vi "DialogCreateInterface.vi"(0 "ClassWriterNative.lvclass":refnum<class "ClassWriterNative.lvclass">, 1 "ProjectItem Refnum":refnum<vi>, 5 "error in (no error)":errorcluster) -> (14 "Reference out":refnum<class "ClassWriterNative.lvclass">, 15 "Cancelled":bool, 16 "CreateInterfaceData":T3, 19 "error out":errorcluster)   [LabVIEW 2020, in "ClassWriterNative.lvclass"]
uses:
  ClassWriterNative.lvclass
  Provider_BaseClassInterface/CreateInterfaceData.ctl
  Provider_BaseClassInterface/ClassWriter_class/InterfaceMethodsToCreate.ctl
  Common/CommonVIs/CommonVIs_AttributeType.ctl
  Common/CommonVIs/CommonVIs_AttributeDataType.ctl
  Common/String/GDSString_AccessScopeModifierType.ctl
  Provider_BaseClassInterface/BaseProvider_SubVIs/BaseProvider_WireList.ctl
  Provider_BaseClassInterface/BaseProvider_SubVIs/BaseProvider_WireStyleType.ctl
  <vilib>/Utility/miscctls.llb/LVRectTypeDef.ctl
  Common/InterfaceLibrary/InterfaceInfo.ctl
  Common/LvClass_class/GDSLvClass_ClassMethodInfo.ctl
  Common/CommonVIs/CommonVIs_ClassIconSelection_Action.ctl
  <vilib>/Utility/miscctls.llb/LVPositionTypeDef.ctl
  <vilib>/Utility/miscctls.llb/LVRowAndColumnUnsignedTypeDef.ctl
  <vilib>/picture/picture.llb/imagedata.ctl
  8226ef7b-d77c-4b82-be33-8974597c5039.vi
  914e6089-59b2-486e-920a-8b2175e33088.vi
  Common/InterfaceLibrary/InterfaceLibrary.lvlib
  Provider_BaseClassInterface/ClassWriter_class/ClassWriter.lvclass
panel:
  out "IconSelection":picture
  in  "WireSelectionList":T1
  out "Wire Style":cluster{"Name":string, "Wire":picture}
  in  "InterfaceFilter":string caption="Filter"
  out "Icon":picture
  in  "_ShowContextHelp":bool
  in  "Help":bool
  in  "ConnectorPanePattern":u16(ring) caption="Connector Pane" items=["4x4x4", "5x6x5", "6x8x6"]
  in  "_UseLLB":bool
  in  "_InterfaceFolderSuffix":string caption="Interface Folder Suffix"
  out "ProductPicture":picture
  out "DupPath":bool
  in  "_InterfaceName":string caption="Interface Name"
  in  "_ClassDescription":string caption="Interface Description"
  in  "_InterfaceFolder":path caption="Save Interface To.."
  out "TriggerSuffixChange":string
  in  "SelectInterfaceClass":i32[](listbox) caption="Select Parent Interface(s) (ctrl+click to do multiple Selection)"
  in  "M":string[][](table)
  out "Over":i32(listbox) caption="Over\nride?"
  out "IconList":i32(listbox)
  in  "Cancel":bool
  in  "CreateInterface":bool
  # "Icon"
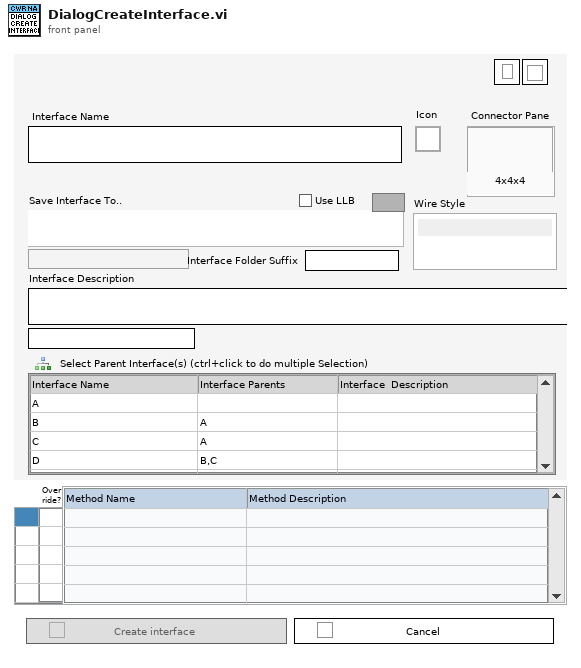
[diagram p1: front panel]
types:
  T1 = typedef "BaseProvider_WireList.ctl" = cluster{"WireStyle":T2[], "WireEditor":bool}
  T2 = typedef "BaseProvider_WireStyleType.ctl" = cluster{"Boolean":bool, "Wire":picture, "Name":string, "Status":u16}
  T3 = typedef "ClassWriter.lvclass/CreateInterfaceData.ctl" = cluster{"InterfaceName":string, "InterfaceFolder":path, "InterfaceDescription":string, "FolderSuffix":string, "MethodsToCreate":T4[], "ParentInterfaces":path[]}
  T4 = typedef "ClassWriter.lvclass/InterfaceMethodsToCreate.ctl" = cluster{"Name":string, "Description":string, "MethodsArgumentsIn":T5[], "MethodsArgumentsOut":T5[], "DecendantsMustOverride":bool}
  T5 = typedef "CommonVIs_AttributeType.ctl" = cluster{"Name":string, "DataType":T6, "ArrayDim":i32, "CtrlPath":path, "DataTypeString":string, "AccessScope":T7, "InitialData":variant}
  T6 = typedef "CommonVIs_AttributeDataType.ctl" = enum16{"UINT8", "INT8", "UINT16", "INT16", "UINT32", "INT32", "UINT64", "INT64", "SGL", "DBL", "EXT", "CSG", "CDB", "CXT", "TimeStamp", "STRING", "PATH", "BOOL", "ENUM", "RefNum", "VIRefNum", "LabVIEW Class", "Cluster", "Variant", "TypeDef", "Waveform", "LabVIEW Object", "Other", "void", "Set", "Map"}
  T7 = typedef "GDSString_AccessScopeModifierType.ctl" = enum16{"public", "private", "protected", "internal"}
  T8 = typedef "LVPositionTypeDef.ctl" = cluster{"Left":i32, "Top":i32}
  T9 = cluster{"Font Name":string, "Size":u16, "Bold":bool, "Italic":bool, "Underline":bool, "Strikeout":bool, "Color":u32}
  T10 = typedef "CommonVIs_ClassIconSelection_Action.ctl" = enum16{"All", "Non Interface", "Only Interface"}
  T11 = typedef "LVRectTypeDef.ctl" = cluster{"Left":i16, "Top":i16, "Right":i16, "Bottom":i16}
  T12 = typedef "InterfaceLibrary.lvlib/InterfaceInfo.ctl" = cluster{"Name(Short if no Conflicts)":string, "FullQualifierName":string, "Description":string, "Path":path, "ParentInterfaceNames(Short if no Conflitcs)":string[], "ParentInterfaceFullQualifierNames":string[], "IconPath":path, "Methods":T13[], "DynamicDispatchMethod":bool[]}
  T13 = typedef "GDSLvClass_ClassMethodInfo.ctl" = cluster{"Name":string, "Descriptions":string, "RelativePath":path, "SourceScope":enum32{"invalid scope", "public", "private", "protected", "community"}, "MustOverride":bool, "VirtualFolderLocation":string[], "DynamicDispatch":bool}
  T14 = cluster{"Cancel":bool, "Derived":bool, "DeriveFromClassRef":refnum<vi>, "InterfacesInList":path[], "DesignPatternsVisible":bool, "ClassProviderName":string, "InitDerived":bool, "ClassFolderSuffix":string, "LLB_Allowed":bool, "StartFolder":path, "SplitterMouseDown":bool, "OldBnds":T11, "BondsChanged":bool, "StartBnds":T11, "InterfaceInfo":T12[], "InterfaceIcons":path[], "ParentInterfaces":path[]}
  T15 = typedef "LVPointTypeDef.ctl" = cluster{"Horizontal":i16, "Vertical":i16}
  T16 = typedef "LVRowAndColumnUnsignedTypeDef.ctl" = cluster{"Row":u32, "Column":u32}
  T17 = enum8{"Enabled", "Disabled", "Disabled and Grayed Out"}
  T18 = typedef "imagedata.ctl" = cluster{"image type":i32, "image depth":i32, "image":u8[], "mask":u8[], "colors":u32[], "Rectangle":cluster{"left":i16, "top":i16, "right":i16, "bottom":i16}}
  T19 = typedef "BaseProvider_IniFileSettings.ctl" = cluster{"ClassFolderSuffix":string, "InterfaceFolderSuffix":string, "InterfaceIcon":string, "FileNamingOption":T20, "DynamicDispatchStartValue":bool}
  T20 = typedef "BaseProvider_FileNamingOption.ctl" = enum16{"CamelCase", "Space", "Underscore"}
  T21 = typedef "Scripting_ConnectorPanePatternType.ctl" = u16
  T22 = enum32{"Invalid", "Standard", "Closed", "Hidden", "Minimized", "Maximized"}
  T23 = typedef "LVPoint32TypeDef.ctl" = cluster{"Horizontal":i32, "Vertical":i32}
  T24 = typedef "GOOP_WireConfigurationType.ctl" = cluster{"Edge thickness":i32, "Edge color":u32, "Center thickness":i32, "Center pattern":T25, "CenterColor1":u32, "CenterColor2":u32, "Tunnels and terminals colors":u32}
  T25 = typedef "GOOP_WirePattern.ctl" = enum16{"Solid", "Large dash", "Small dash"}
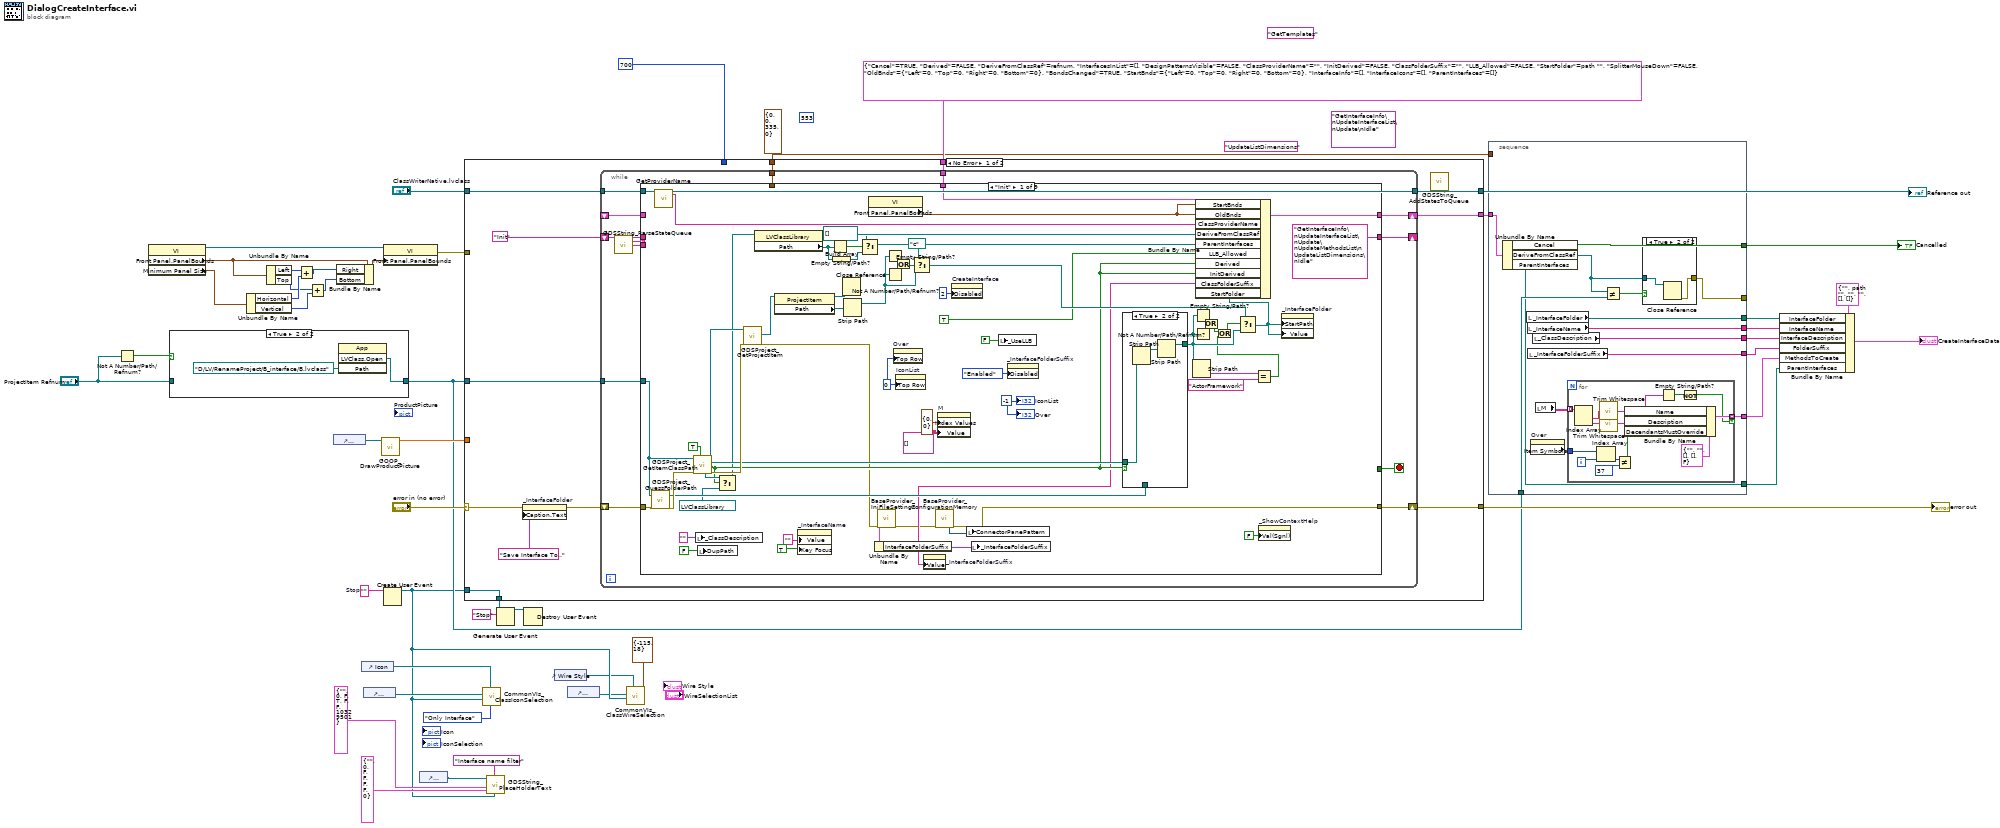
[diagram p0: block diagram]
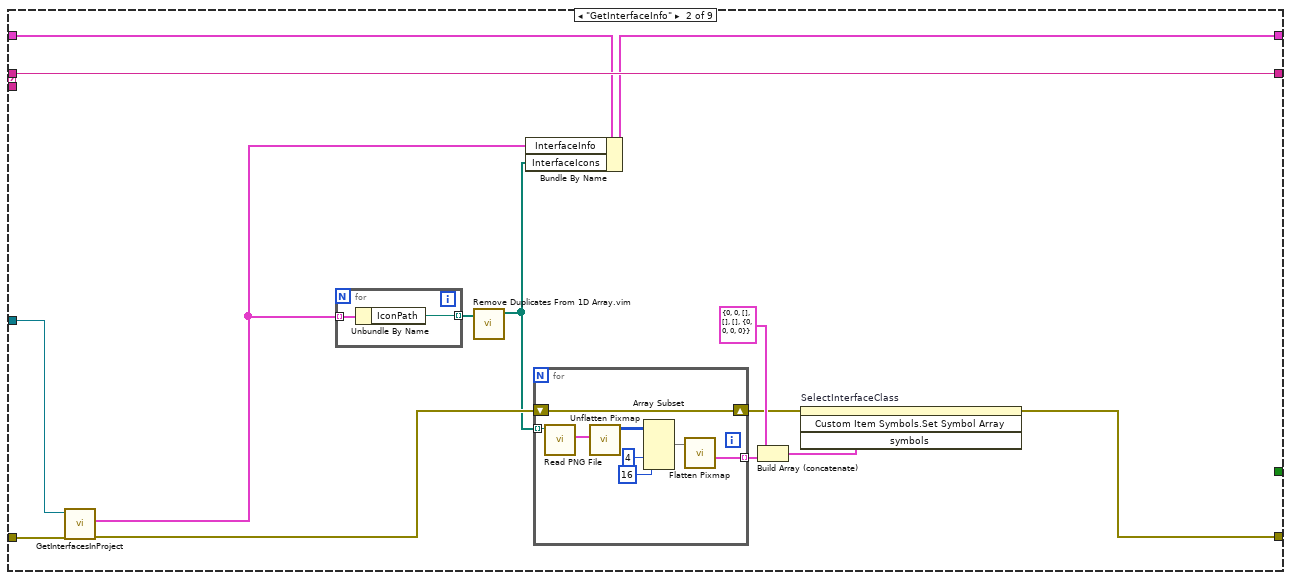
[diagram p5: hidden frame]
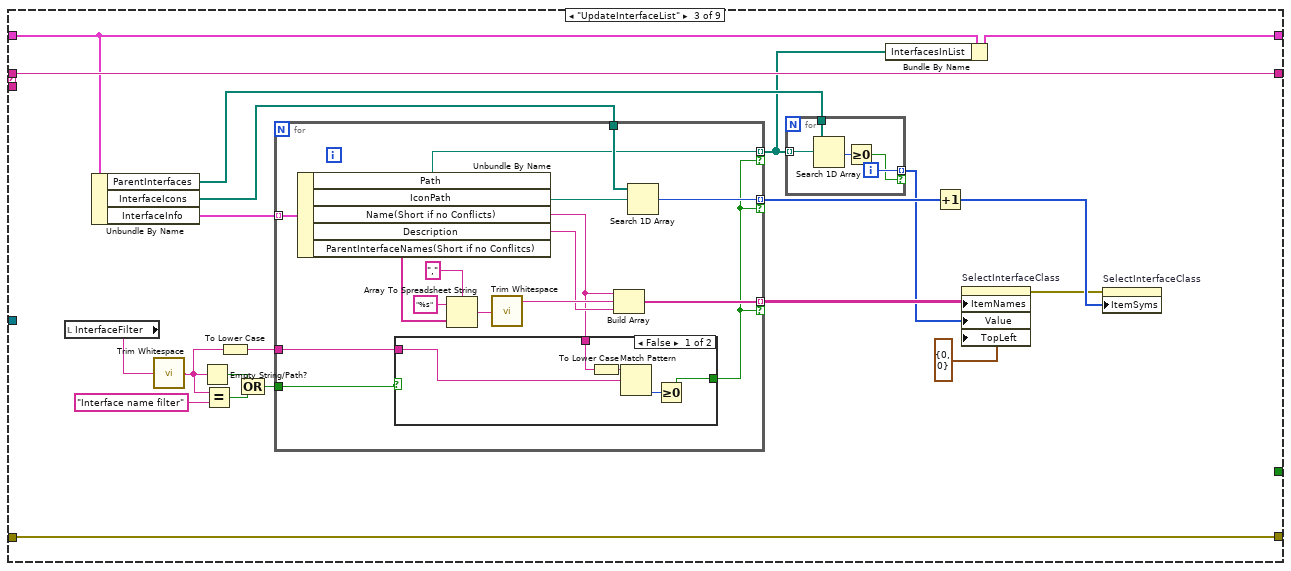
[diagram p6: hidden frame]
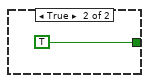
[diagram p7: hidden frame]
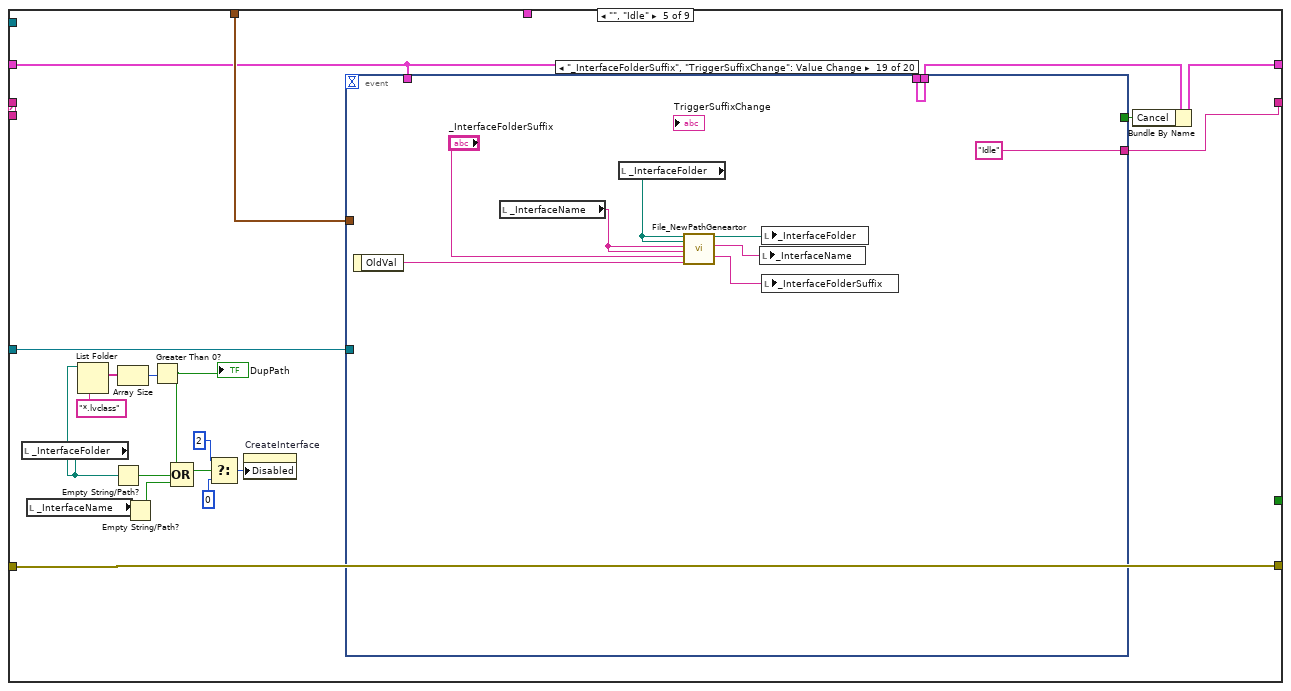
[diagram p9: hidden frame]
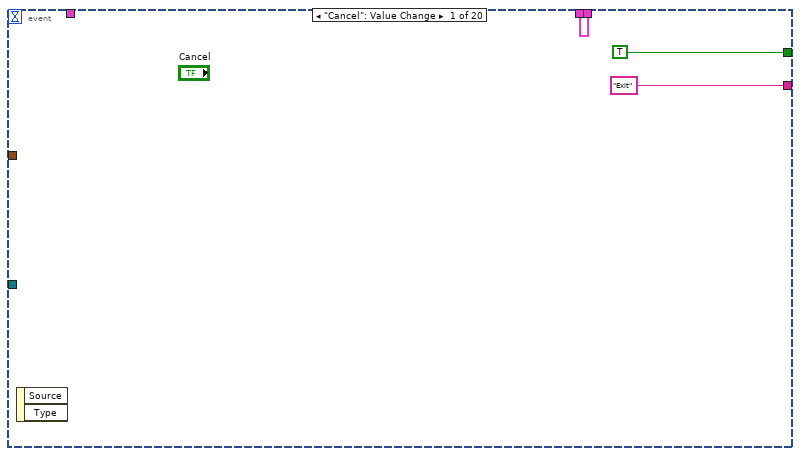
[diagram p10: hidden frame]
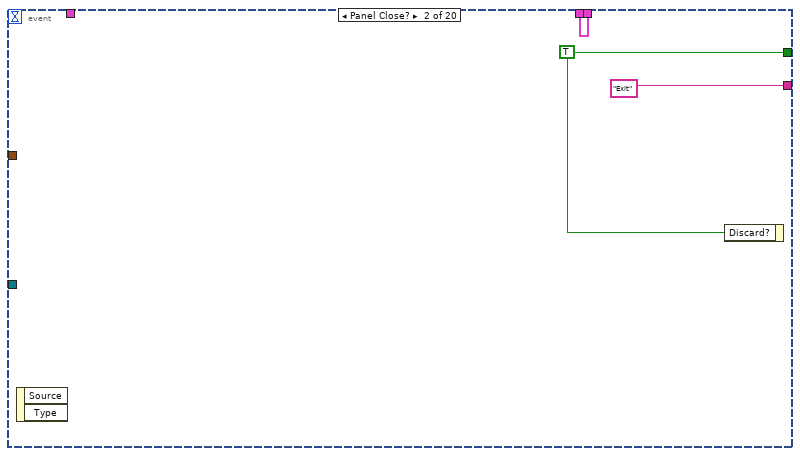
[diagram p11: hidden frame]
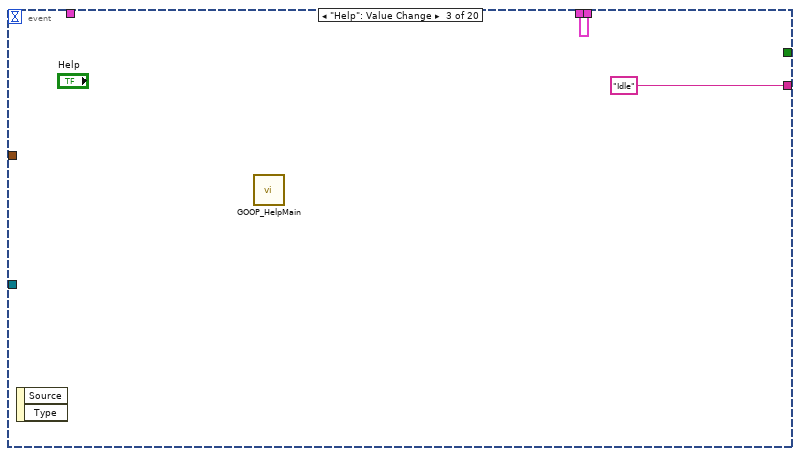
[diagram p12: hidden frame]
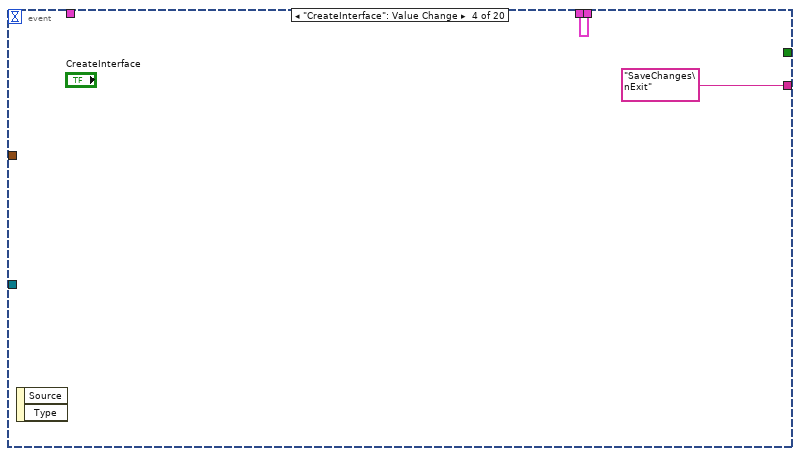
[diagram p13: hidden frame]
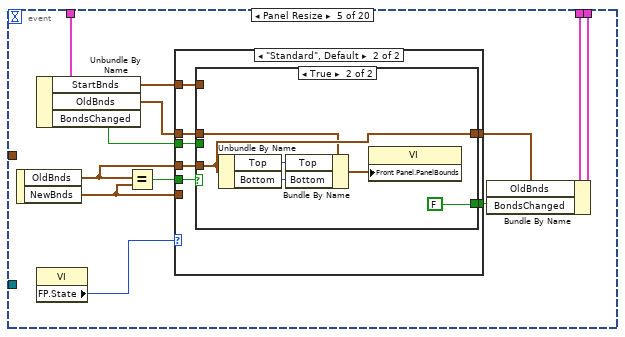
[diagram p14: hidden frame]
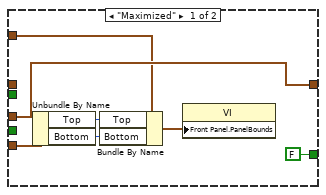
[diagram p15: hidden frame]
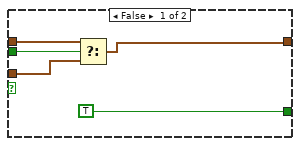
[diagram p16: hidden frame]
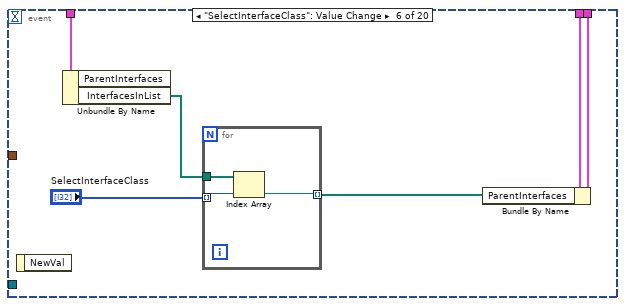
[diagram p17: hidden frame]
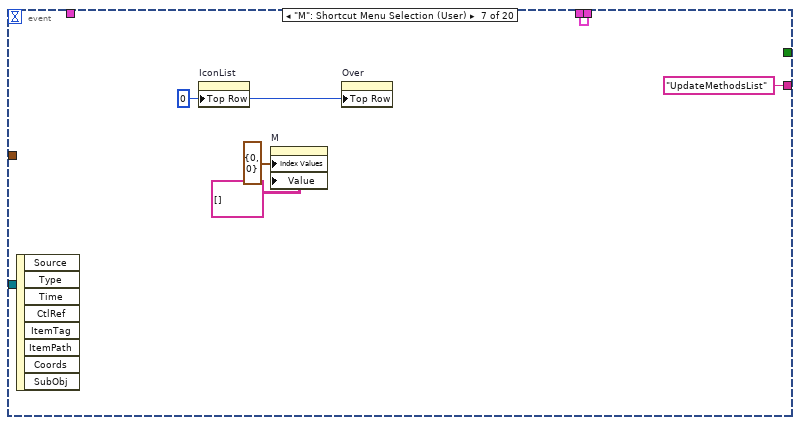
[diagram p18: hidden frame]
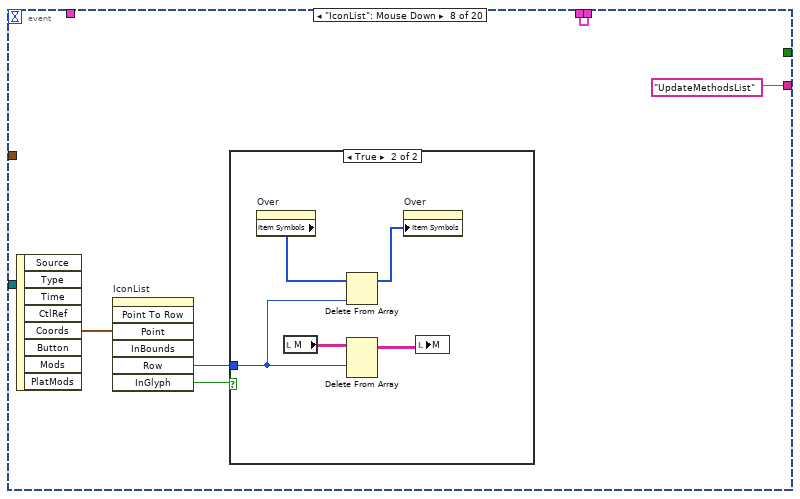
[diagram p19: hidden frame]
diagram:
  (unwired) "UpdateListDimensions"
  w6 = ""  # Stop
  (unwired) "GetInterfaceInfo\nUpdateInterfaceList\nUpdate\nIdle"
  (unwired) i16 553 ("Right")
  w38 = T11 {"Left"=0, "Top"=0, "Right"=335, "Bottom"=0} ("Rect")
  (unwired) "GetTemplates"
  n1 = Not A Number/Path/Refnum?(number/path/refnum="ProjectItem Refnum") -> (NaN/Path/Refnum?=w18:bool)
  n2 = property class="VI"() -> (reference out=w34:refnum<vi>, "Front Panel.PanelBounds"=w32:T11, "Minimum Panel Size"=w30:T15)  [unwired: 2 in, 1 out]
  n3 = case shown="True" w18 {
    tunnel: "ProjectItem Refnum" -> [w49 _]
    tunnel: [w49 w50] -> w16
    frame False {
    }
    frame True {
      n4 = invoke class="App" method="LVClass.Open"("Path"=path "D:/LV/RenameProject/B_interface/B.lvclass") -> ("LVClass.Open"=w50:refnum<vi>)  [unwired: 3 in, 3 out]
    }
  }
  n5 = Unbundle By Name(w30) -> ("Horizontal"=w29:i16, "Vertical"=w26:i16)
  n6 = Unbundle By Name(w32) -> ("Left"=w31:i16, "Top"=w27:i16)
  n7 = Add(x=w31, y=w29) -> (x+y=w28:i16)
  n8 = Add(x=w27, y=w26) -> (x+y=w25:i16)
  n9 = control-ref of="ProductPicture"() -> (w36:refnum<vi>)
  n10 = Bundle By Name(cluster=w32, "Right"=w28, "Bottom"=w25) -> (w33:T11)
  n11 = control-ref of="Icon"() -> (w22:refnum<vi>)
  n12 = control-ref of="IconSelection"() -> (w21:refnum<vi>)
  n13 = call "GOOP_DrawProductPicture.vi"("ProductPictureControl"=w36) -> ("Zoom Factor"=w35:sgl)  [unwired: 10 in]
  n14 = Create User Event(user event datatype=w6) -> (user event=w3:refnum<user-event>)  [unwired: 1 in, 1 out]
  n15 = property class="VI"(reference=w34, "Front Panel.PanelBounds"=w33) -> (error out=w24:errorcluster)  [unwired: 1 in, 1 out]
  n16 = control-ref of="InterfaceFilter"() -> (w7:refnum<vi>)
  n17 = case shown="No Error" "error in (no error)" {
    selector: "error in (no error)" -> [w55 w431]
    tunnel: "ClassWriterNative.lvclass" -> [w61 w430]
    tunnel: [w53 w431] -> w47
    tunnel: [w62 w430] -> w45
    tunnel: T14 {"Cancel"=TRUE, "Derived"=FALSE, "DeriveFromClassRef"=refnum, "InterfacesInList"=[], "DesignPatternsVisible"=FALSE, "ClassProviderName"="", "InitDerived"=FALSE, "ClassFolderSuffix"="", "LLB_Allowed"=FALSE, "StartFolder"=path "", "SplitterMouseDown"=FALSE, "OldBnds"={"Left"=0, "Top"=0, "Right"=0, "Bottom"=0}, "BondsChanged"=TRUE, "StartBnds"={"Left"=0, "Top"=0, "Right"=0, "Bottom"=0}, "InterfaceInfo"=[], "InterfaceIcons"=[], "ParentInterfaces"=[]} ("output cluster") -> [w60 _]
    tunnel: w16 -> [w59 _]
    tunnel: [w58 _] -> w43
    tunnel: w38 -> [w57 _]
    tunnel: w35 -> [_ _]
    tunnel: w24 -> [_ _]
    tunnel: [w52 w429] -> w19
    tunnel: w3 -> [w52 w429]
    tunnel: 700 ("Splitter Position") -> [_ _]
    frame No Error {
      n18 = property on="_InterfaceFolder" class="Path"(error in=w55, "Caption.Text"="Save Interface To.." ("t")) -> (error out=w56:errorcluster)  [unwired: 1 in, 1 out]
      n19 = while {
        shift-right: [w75] -> w53
        shift-left: w56 -> [w77]
        shift-right: [w65] -> _
        shift-left: "Init" -> [w69]
        shift-right: [w71] -> w58
        shift-left: _ -> [w76]
        tunnel: w61 -> [w74]
        tunnel: [w74] -> w62
        tunnel: w60 -> [w73]
        tunnel: w59 -> [w72]
        tunnel: w57 -> [w70]
        stop <- w64 stop-if-true
        n20 = call "GDSString_ParseStateQueue.vi"("State Queue"=w69) -> ("Remaining States"=w67:string, "Current State"=w68:string, "Arguments"=w66:string)  [unwired: 10 in, 2 out]
        n21 = case shown="\"Init\"" w68 {
          tunnel: w76 -> [_ w153 w169 w215 w216 w392 w415 w422 w428]
          tunnel: [w135 w150 w166 w215 w232 w392 w415 w422 w428] -> w71
          tunnel: w77 -> [w119 w152 w185 w213 w235 w391 w414 w421 w425]
          tunnel: [w92 w143 w185 w213 w235 w391 w414 w421 w425] -> w75
          tunnel: w74 -> [w113 _ _ _ _ _ _ _ _]
          tunnel: ["GetInterfaceInfo\nUpdateInterfaceList\nUpdate\nUpdateMethodsList\n UpdateListDimensions\nIdle" w154 w184 w214 w233 w390 w413 w420 "Exit"] -> w65
          tunnel: w73 -> [w134 _ _ _ _ _ _ _ _]
          tunnel: w72 -> [w117 w151 _ _ w219 _ _ _ _]
          tunnel: w70 -> [_ _ _ _ w217 _ _ _ _]
          tunnel: w67 -> [_ w154 w184 w214 _ w390 w413 w420 _]
          tunnel: w66 -> [_ _ _ _ _ _ _ _ _]
          tunnel: [_ _ _ _ _ _ _ _ TRUE] -> w64
          frame "Init" {
            w78 = -1 ("IconList")
            w79 = 0 ("Top Row")
            n22 = call "GDSProject_GuessFolderPath.vi"("ProjectItem"=w117, "error in (no error)"=w119) -> ("Path"=w116:path, "error out"=w118:errorcluster)  [unwired: 14 in, 2 out]
            n23 = call-dynamic "GetProviderName.vi"("ClassWriterNative in"=w113) -> ("ProviderName"=w106:string)  [unwired: 15 in, 3 out]
            n24 = call "GDSProject_GetItemClassPath.vi"("ReturnRefToClass(False)"=TRUE, "error in"=w118, "ProjectItemRefIn"=w117) -> ("error out"=w132:errorcluster, "LvCLassFound"=w108:bool, "Path"=w114:path, "ProjectItemRefOut"=w131:refnum<vi>, "LvClassRef"=w110:refnum<vi>)  [unwired: 3 in, 1 out]
            n25 = local write "_ClassDescription"("" ("Class description")) -> ()
            n26 = local write "DupPath"(FALSE ("DupPath")) -> ()
            n27 = Select(t=w110, s=w108, f=refnum<vi> refnum) -> (s? t:f=w88:refnum<vi>)
            n28 = call "GDSProject_GetProjectItem.vi"("ProjectItemToSearchFrom"=w131, "error in (no error)"=w132) -> ("ProjectItemFound"=w87:refnum<vi>, "error out"=w93:errorcluster)  [unwired: 14 in, 2 out]
            n29 = property class="LVClassLibrary"(reference=w88) -> ("Path"=w85:path)  [unwired: 1 in, 2 out]
            n30 = property class="ProjectItem"(reference=w87) -> (reference out=w89:refnum<vi>, "Path"=w121:path)  [unwired: 1 in, 1 out]
            n31 = property on="_InterfaceName" class="Str"("Value"="" ("Class name"), "Key Focus"=TRUE) -> ()  [unwired: 2 in, 2 out]
            n32 = Empty String/Path?(string/path=w85) -> (empty?=w86:bool)
            n33 = Build Array(w85) -> (w84:path[])
            n34 = Close Reference(reference=w89) -> ()  [unwired: 1 in, 1 out]
            n35 = Strip Path(path=w121) -> (stripped path=w120:path)  [unwired: 1 out]
            n36 = Select(t=path[] [], s=w86, f=w84) -> (s? t:f=w82:path[])
            n37 = property class="VI"() -> ("Front Panel.PanelBounds"=w90:T11)  [unwired: 2 in, 2 out]
            n38 = call "BaseProvider_IniFileSettings.vi"("error in (no error)"=w93) -> ("IniFileSettings"=w107:T19)  [unwired: 17 in, 1 out]
            n39 = Unbundle By Name(w107) -> ("InterfaceFolderSuffix"=w105:string)
            n40 = Empty String/Path?(string/path=w120) -> (empty?=w122:bool)
            n41 = Not A Number/Path/Refnum?(number/path/refnum=w120) -> (NaN/Path/Refnum?=w123:bool)
            n42 = property on="Over" class="LstBox (strict)"("Top Row"=w79) -> ()  [unwired: 2 in, 2 out]
            n43 = Or(x=w122, y=w123) -> (x .or. y?=w124:bool)
            n44 = property on="IconList" class="LstBox (strict)"("Top Row"=w79) -> ()  [unwired: 2 in, 2 out]
            n45 = Select(t=path "c:/", s=w124, f=w120) -> (s? t:f=w111:path)
            n46 = property on="_InterfaceFolderSuffix" class="Str"("Value"=w105) -> ()  [unwired: 2 in, 2 out]
            n47 = call "BaseProvider_ConfigurationMemory.vi"("error in (no error)"=w93) -> ("PatternOut"=w91:T21, "error out"=w92:errorcluster)  [unwired: 12 in, 5 out]
            n48 = property on="M" class="Tbl (strict)"("Index Values"=T16 {"Row"=0, "Column"=0}, "Value"=string[][] [] ("Methods")) -> ()  [unwired: 2 in, 2 out]
            n49 = property on="CreateInterface" class="Bool"("Disabled"=u8 2) -> ()  [unwired: 2 in, 2 out]
            n50 = local write "ConnectorPanePattern"(w91) -> ()
            n51 = local write "_InterfaceFolderSuffix"(w105) -> ()
            n52 = local write "_UseLLB"(FALSE ("_UseLLB")) -> ()
            n53 = property on="_InterfaceFolderSuffix" class="Str"("Disabled"=T17."Enabled") -> ()  [unwired: 2 in, 2 out]
            n54 = case shown="True" w108 {
              tunnel: w114 -> [_ w140]
              tunnel: [w137 w138] -> w103
              tunnel: w116 -> [w137 _]
              frame False {
              }
              frame True {
                n55 = Strip Path(path=w140) -> (stripped path=w139:path)  [unwired: 1 out]
                n56 = Strip Path(path=w139) -> (stripped path=w138:path)  [unwired: 1 out]
              }
            }
            n57 = Strip Path(path=w103) -> (name=w102:string)  [unwired: 1 out]
            n58 = Empty String/Path?(string/path=w103) -> (empty?=w127:bool)
            n59 = Not A Number/Path/Refnum?(number/path/refnum=w103) -> (NaN/Path/Refnum?=w126:bool)
            n60 = Or(x=w127, y=w126) -> (x .or. y?=w100:bool)
            n61 = Equal?(x=w102, y="ActorFramework") -> (x = y?=w99:bool)
            n62 = Or(x=w100, y=w99) -> (x .or. y?=w98:bool)
            n63 = Select(t=w111, s=w98, f=w103) -> (s? t:f=w104:path)
            n64 = Bundle By Name(cluster=w134, "StartBnds"=w90, "OldBnds"=w90, "ClassProviderName"=w106, "DeriveFromClassRef"=w88, "ParentInterfaces"=w82, "LLB_Allowed"=TRUE, "Derived"=w108, "InitDerived"=w108, "ClassFolderSuffix"=w105, "StartFolder"=w104) -> (w135:T14)
            n65 = property on="_ShowContextHelp" class="Bool (strict)"("Val(Sgnl)"=FALSE ("Value (Signaling)")) -> ()  [unwired: 2 in, 2 out]
            n66 = property on="_InterfaceFolder" class="Path"("StartPath"=w104, "Value"=w104) -> ()  [unwired: 2 in, 2 out]
            "IconList" <- w78
            "Over" <- w78
          }
          frame "GetInterfaceInfo" {
            n67 = call "GetInterfacesInProject.vi"("error in"=w152, "Project/ProjectItem"=w151) -> ("error out"=w144:errorcluster, "InterfaceInfo"=w142:T12[])  [unwired: 8 in]
            n68 = for {
              tunnel: w142 -> [w164] mode=indexing
              tunnel: [w163] -> w145 mode=indexing
              n69 = Unbundle By Name(w164) -> ("IconPath"=w163:path)
            }
            n70 = call "Remove Duplicates From 1D Array.vim"("array"=w145) -> ("array with duplicates removed"=w141:path[])  [unwired: 10 in]
            n71 = Bundle By Name(cluster=w153, "InterfaceInfo"=w142, "InterfaceIcons"=w141) -> (w150:T14)
            n72 = for {
              tunnel: w141 -> [w162] mode=indexing
              shift-right: [w156] -> w146
              shift-left: w144 -> [w156]
              tunnel: [w155] -> w147 mode=indexing
              n73 = call <vilib>:"Read PNG File.vi"("path to PNG file"=w162) -> ("image data"=w161:T18)  [unwired: 8 in, 2 out]
              n74 = call <vilib>:"Unflatten Pixmap.vi"("image data"=w161) -> ("24-bit pixmap"=w160:u32[][])  [unwired: 4 in, 6 out]
              n75 = Array Subset(array=w160, index (col)=4 ("index"), length (col)=16 ("length")) -> (w157:u32[][])  [unwired: 2 in]
              n76 = call <vilib>:"Flatten Pixmap.vi"("24-bit pixmap"=w157) -> ("image data"=w155:T18)  [unwired: 10 in]
            }
            n77 = Build Array (concatenate)(T18 {"image type"=0, "image depth"=0, "image"=[], "mask"=[], "colors"=[], "Rectangle"={"left"=0, "top"=0, "right"=0, "bottom"=0}} ("image data"), w147) -> (w149:T18[])
            n78 = invoke on="SelectInterfaceClass" class="MCListbox (strict)" method="Custom Item Symbols.Set Symbol Array"(error in=w146, "symbols"=w149) -> (error out=w143:errorcluster)  [unwired: 2 in, 3 out]
          }
          frame "UpdateInterfaceList" {
            n79 = local read "InterfaceFilter"() -> (w170:string)
            n80 = Unbundle By Name(w169) -> ("ParentInterfaces"=w168:path[], "InterfaceIcons"=w172:path[], "InterfaceInfo"=w171:T12[])
            n81 = call <vilib>:"Trim Whitespace.vi"("string"=w170) -> ("trimmed string"=w179:string)  [unwired: 1 in]
            n82 = Empty String/Path?(string/path=w179) -> (empty?=w176:bool)
            n83 = Equal?(x=w179, y="Interface name filter" ("InterfaceFilter")) -> (x = y?=w177:bool)
            n84 = To Lower Case(string=w179) -> (all lower case string=w181:string)
            n85 = Compound Arithmetic op=OR(w176, w177) -> (w178:bool)
            n86 = for {
              tunnel: [w202] -> w173 mode=indexing if=w191
              tunnel: w171 -> [w201] mode=indexing
              tunnel: w172 -> [w197]
              tunnel: [w196] -> w182 mode=indexing if=w191
              tunnel: w178 -> [w195]
              tunnel: w181 -> [w193]
              tunnel: [w192] -> w165 mode=indexing if=w191
              n87 = Unbundle By Name(w201) -> ("Path"=w192:path, "IconPath"=w198:path, "Name(Short if no Conflicts)"=w194:string, "Description"=w199:string, "ParentInterfaceNames(Short if no Conflitcs)"=w200:string[])
              n88 = case shown="False" w195 {
                tunnel: [w208 TRUE] -> w191
                tunnel: w194 -> [w211 _]
                tunnel: w193 -> [w210 _]
                frame False {
                  n89 = To Lower Case(string=w211) -> (all lower case string=w207:string)
                  n90 = Match Pattern(string=w207, regular expression=w210) -> (offset past match=w209:i32)  [unwired: 1 in, 3 out]
                  n91 = Greater Or Equal To 0?(x=w209) -> (x >= 0?=w208:bool)
                }
                frame True {
                }
              }
              n92 = Array To Spreadsheet String(delimiter (Tab)=",", array=w200, 3:"%s" ("format string")) -> (spreadsheet string=w204:string)
              n93 = call <vilib>:"Trim Whitespace.vi"("string"=w204) -> ("trimmed string"=w203:string)  [unwired: 1 in]
              n94 = Build Array(w194, w203, w199) -> (w202:string[])
              n95 = Search 1D Array(1D array=w197, element=w198) -> (index of element=w196:i32)  [unwired: 1 in]
            }
            n96 = for {
              tunnel: w165 -> [w190] mode=indexing
              tunnel: w168 -> [w189]
              tunnel: [w187] -> w167 mode=indexing if=w186
              i -> [w187]
              n97 = Search 1D Array(1D array=w189, element=w190) -> (index of element=w188:i32)  [unwired: 1 in]
              n98 = Greater Or Equal To 0?(x=w188) -> (x >= 0?=w186:bool)
            }
            n99 = Bundle By Name(cluster=w169, "InterfacesInList"=w165) -> (w166:T14)
            n100 = Increment(x=w182) -> (x+1=w183:i32[])
            n101 = property on="SelectInterfaceClass" class="MCListbox (strict)"("ItemNames"=w173, "Value"=w167, "TopLeft"=T16 {"Row"=0, "Column"=0} ("Top Left Visible Cell")) -> (error out=w174:errorcluster)  [unwired: 2 in, 1 out]
            n102 = property on="SelectInterfaceClass" class="MCListbox (strict)"(error in=w174, "ItemSyms"=w183) -> ()  [unwired: 1 in, 2 out]
          }
          frame "Update" {
          }
          frame "", "Idle" {
            n103 = local read "_InterfaceFolder"() -> (w224:path)
            n104 = local read "_InterfaceName"() -> (w225:string)
            n105 = List Folder(path=w224, pattern="*.lvclass") -> (filenames=w222:string[])  [unwired: 2 in, 3 out]
            n106 = Empty String/Path?(string/path=w224) -> (empty?=w227:bool)
            n107 = Array Size(array=w222) -> (size(s)=w221:i32)
            n108 = Empty String/Path?(string/path=w225) -> (empty?=w226:bool)
            n109 = Greater Than 0?(x=w221) -> (x > 0?=w220:bool)
            "DupPath" <- w220
            n110 = Compound Arithmetic op=OR(w220, w227, w226) -> (w228:bool)
            n111 = Select(t=u8 2, s=w228, f=u8 0 ("Disabled")) -> (s? t:f=w231:u8)
            n112 = property on="CreateInterface" class="Bool"("Disabled"=w231) -> ()  [unwired: 2 in, 2 out]
            n113 = event shown="[18] \"_InterfaceFolderSuffix\", \"TriggerSuffixChange\": Value Change" {
              selector: _ -> [_ _ _ _ _ _ _ _ _ _ _ _ _ _ _ _ _ _ _ _]
              dyn-events: _ -> [_ _ _ _ _ _ _ _ _ _ _ _ _ _ _ _ _ _ _ _]
              timeout: _ -> [_ _ _ _ _ _ _ _ _ _ _ _ _ _ _ _ _ _ _ _]
              tunnel: ["Exit" "Exit" "Idle" "SaveChanges\nExit" _ _ "UpdateMethodsList" "UpdateMethodsList" "UpdateListDimensions" "UpdateMethodsList" "UpdateMethodsList" _ _ "Idle" "UpdateInterfaceList" "Idle" "Idle" "Idle" "Idle" "Idle"] -> w233
              tunnel: [TRUE w240 _ _ _ _ _ _ _ _ _ _ _ _ _ _ _ _ _ _] -> w234
              tunnel: w216 -> [_ _ _ _ w252 w286 _ _ _ _ _ _ _ _ _ _ _ _ _ _]
              tunnel: w219 -> [_ _ _ _ _ _ _ _ _ _ _ _ _ _ _ _ _ _ _ _]
              tunnel: w216 -> [w236 w239 w242 w244 w251 w288 w296 w301 w308 w313 w322 w326 w332 w333 w336 w347 w349 w357 w366 w375]
              tunnel: [w236 w239 w242 w244 w250 w284 w296 w301 w308 w313 w322 w326 w332 w333 w336 w347 w349 w357 w366 w375] -> w218
              tunnel: w217 -> [_ _ _ _ _ _ _ _ _ _ _ _ _ _ _ _ _ _ _ _]
              event "Cancel": Value Change {
                n114 = event-data() -> ()  [unwired: 1 in, 2 out]
              }
              event Panel Close? {
                w240 = TRUE
                n115 = event-data() -> ()  [unwired: 1 in, 2 out]
                n116 = event-data("Discard?"=w240) -> ()  [unwired: 1 in, 1 out]
              }
              event "Help": Value Change {
                n117 = event-data() -> ()  [unwired: 1 in, 2 out]
                n118 = call "GOOP_HelpMain.vi"() -> ()  [unwired: 12 in]
              }
              event "CreateInterface": Value Change {
                n119 = event-data() -> ()  [unwired: 1 in, 2 out]
              }
              event Panel Resize {
                n120 = event-data() -> ("OldBnds"=w249:T11, "NewBnds"=w247:T11)  [unwired: 1 in]
                n121 = Unbundle By Name(w252) -> ("StartBnds"=w246:T11, "OldBnds"=w254:T11, "BondsChanged"=w256:bool)
                n122 = property class="VI"() -> ("FP.State"=w248:T22)  [unwired: 2 in, 2 out]
                n123 = Equal?(x=w249, y=w247) -> (x = y?=w253:bool)
                n124 = case shown="\"Standard\", Default" w248 {
                  tunnel: [w259 w271] -> w257
                  tunnel: w256 -> [_ w270]
                  tunnel: [FALSE w269] -> w255
                  tunnel: w254 -> [_ w268]
                  tunnel: w253 -> [_ w267]
                  tunnel: w249 -> [w259 w266]
                  tunnel: w247 -> [w262 _]
                  tunnel: w246 -> [w258 w265]
                  frame "Maximized" {
                    n125 = Unbundle By Name(w262) -> ("Top"=w264:i16, "Bottom"=w263:i16)
                    n126 = Bundle By Name(cluster=w258, "Top"=w264, "Bottom"=w263) -> (w261:T11)
                    n127 = property class="VI"("Front Panel.PanelBounds"=w261) -> ()  [unwired: 2 in, 2 out]
                  }
                  frame "Standard", Default {
                    n128 = case shown="True" w267 {
                      tunnel: w266 -> [w273 w278]
                      tunnel: [w274 w278] -> w271
                      tunnel: w268 -> [w275 w277]
                      tunnel: [TRUE FALSE] -> w269
                      tunnel: w270 -> [w272 _]
                      tunnel: w265 -> [_ _]
                      frame False {
                        n129 = Select(t=w275, s=w272, f=w273) -> (s? t:f=w274:T11)
                      }
                      frame True {
                        n130 = Unbundle By Name(w278) -> ("Top"=w282:i16, "Bottom"=w281:i16)
                        n131 = Bundle By Name(cluster=w277, "Top"=w282, "Bottom"=w281) -> (w280:T11)
                        n132 = property class="VI"("Front Panel.PanelBounds"=w280) -> ()  [unwired: 2 in, 2 out]
                      }
                    }
                  }
                }
                n133 = Bundle By Name(cluster=w251, "OldBnds"=w257, "BondsChanged"=w255) -> (w250:T14)
              }
              event "SelectInterfaceClass": Value Change {
                n134 = event-data() -> ()  [unwired: 1 in, 1 out]
                n135 = Unbundle By Name(w286) -> ("InterfacesInList"=w285:path[])  [unwired: 1 out]
                n136 = for {
                  tunnel: "SelectInterfaceClass" -> [w290] mode=indexing
                  tunnel: w285 -> [w291]
                  tunnel: [w289] -> w283 mode=indexing
                  n137 = Index Array(array=w291, index=w290) -> (element=w289:path)
                }
                n138 = Bundle By Name(cluster=w288, "ParentInterfaces"=w283) -> (w284:T14)
              }
              event "M": Shortcut Menu Selection (User) {
                w292 = 0 ("Top Row")
                n139 = event-data() -> ()  [unwired: 1 in, 8 out]
                n140 = property on="IconList" class="LstBox (strict)"("Top Row"=w292) -> ()  [unwired: 2 in, 2 out]
                n141 = property on="M" class="Tbl (strict)"("Index Values"=T16 {"Row"=0, "Column"=0}, "Value"=string[][] [] ("Methods")) -> ()  [unwired: 2 in, 2 out]
                n142 = property on="Over" class="LstBox (strict)"("Top Row"=w292) -> ()  [unwired: 2 in, 2 out]
              }
              event "IconList": Mouse Down {
                n143 = event-data() -> ("Coords"=w300:T23)  [unwired: 1 in, 7 out]
                n144 = invoke on="IconList" class="LstBox (strict)" method="Point To Row"("Point"=w300) -> ("Row"=w298:i32, "InGlyph"=w299:bool)  [unwired: 6 in, 5 out]
                n145 = case shown="True" w299 {
                  tunnel: w298 -> [_ w304]
                  frame False {
                  }
                  frame True {
                    n146 = property on="Over" class="LstBox (strict)"() -> ("Item Symbols"=w303:i32[])  [unwired: 2 in, 2 out]
                    n147 = local read "M"() -> (w306:string[][])
                    n148 = Delete From Array(array=w303, index=w304) -> (array with subset deleted=w302:i32[])  [unwired: 1 in, 1 out]
                    n149 = Delete From Array(array=w306, index (row)=w304) -> (array with subset deleted=w305:string[][])  [unwired: 2 in, 1 out]
                    n150 = property on="Over" class="LstBox (strict)"("Item Symbols"=w302) -> ()  [unwired: 2 in, 2 out]
                    n151 = local write "M"(w305) -> ()
                  }
                }
              }
              event Pane Size {
                n152 = event-data() -> ()  [unwired: 1 in, 6 out]
              }
              event "Over": Mouse Down {
                n153 = event-data() -> ("Coords"=w312:T23)  [unwired: 1 in, 7 out]
                n154 = invoke on="Over" class="LstBox (strict)" method="Point To Row"("Point"=w312) -> ("Row"=w310:i32, "InGlyph"=w311:bool)  [unwired: 6 in, 5 out]
                n155 = case shown="True" w311 {
                  tunnel: w310 -> [_ w315]
                  frame False {
                  }
                  frame True {
                    n156 = property on="Over" class="LstBox (strict)"() -> ("Item Symbols"=w314:i32[])  [unwired: 2 in, 2 out]
                    n157 = Index Array(array=w314) -> (element=w317:i32)  [unwired: 1 in]
                    n158 = case shown="0, Default" w317 {
                      tunnel: [37 38] -> w318
                      frame 0, Default {
                      }
                      frame 37 {
                      }
                    }
                    n159 = Replace Array Subset(array=w314, new element=w318, index=w315) -> (w316:i32[])
                    n160 = property on="Over" class="LstBox (strict)"("Item Symbols"=w316) -> ()  [unwired: 2 in, 2 out]
                  }
                }
              }
              event "M": Value Change {
                n161 = event-data() -> ()  [unwired: 1 in, 6 out]
              }
              event "M": Mouse Move; "M": Mouse Wheel {
                n162 = event-data() -> ()  [unwired: 1 in, 5 out]
                n163 = property on="M" class="Tbl (strict)"() -> ("Index Values"=w325:T16)  [unwired: 2 in, 2 out]
                n164 = Unbundle By Name(w325) -> ("Row"=w323:u32)
                n165 = call "Is Value Changed.vim"("value"=w323) -> ("changed or first call?"=w324:bool)
                n166 = case shown="True" w324 {
                  tunnel: w323 -> [_ w327]
                  frame False {
                  }
                  frame True {
                    n167 = property on="IconList" class="LstBox (strict)"("Top Row"=w327) -> ()  [unwired: 2 in, 2 out]
                    n168 = property on="Over" class="LstBox (strict)"("Top Row"=w327) -> ()  [unwired: 2 in, 2 out]
                  }
                }
              }
              event "ConnectorPanePattern": Value Change {
                n169 = event-data() -> ()  [unwired: 1 in, 6 out]
                n170 = call "BaseProvider_ConfigurationMemory.vi"() -> ("WireConfigurationOut"=w330:T24, "IconOut"=w331:string)  [unwired: 13 in, 5 out]
                n171 = call "BaseProvider_ConfigurationMemory.vi"("WireConfiguration"=w330, "Icon"=w331, "Action"=enum16{"Read", "Load", "Save", "Set"}."Save", "PatternIn"="ConnectorPanePattern") -> ()  [unwired: 9 in, 7 out]
              }
              event "_ClassDescription": Value Change {
                n172 = event-data() -> ()  [unwired: 1 in, 2 out]
              }
              event "InterfaceFilter": Value Change {
                n173 = event-data() -> ()  [unwired: 1 in, 6 out]
              }
              event "_InterfaceName": Value Change {
                n174 = event-data() -> ("OldVal"=w345:string)  [unwired: 1 in]
                n175 = local read "_InterfaceFolderSuffix"() -> (w342:string)
                n176 = local read "_UseLLB"() -> (w343:bool)
                n177 = Select(t=".llb", s=w343, f=w342) -> (s? t:f=w341:string)
                n178 = local read "_InterfaceFolder"() -> (w340:path)
                n179 = call "File_NewPathGeneartor.vi"("NewPath"=w340, "OldPath"=w340, "NewName"="_InterfaceName", "OldName"=w345, "NewSuffix"=w342, "OldSuffix"=w341) -> ("PathOut"=w339:path, "NameOut"=w338:string, "SuffixOut"=w337:string)  [unwired: 11 in]
                n180 = local write "_InterfaceName"(w338) -> ()
                n181 = local write "_InterfaceFolderSuffix"(w337) -> ()
                n182 = local write "_InterfaceFolder"(w339) -> ()
              }
              event "_UseLLB": Value Change {
                n183 = event-data() -> ()  [unwired: 1 in, 2 out]
                n184 = Select(t=u8 2 ("Disabled"), s="_UseLLB", f=u8 0 ("Disabled")) -> (s? t:f=w353:u8)
                n185 = property on="_InterfaceName" class="Str"() -> ("Value"=w350:string)  [unwired: 2 in, 2 out]
                n186 = property on="_InterfaceFolderSuffix" class="Str"("Disabled"=w353) -> ()  [unwired: 2 in, 2 out]
                n187 = property on="_InterfaceName" class="Str"("Val(Sgnl)"=w350) -> ()  [unwired: 2 in, 2 out]
              }
              event "_ShowContextHelp": Value Change {
                n188 = event-data() -> ("NewVal"=w356:bool)  [unwired: 1 in]
                n189 = Control Help Window(1:w356) -> ()  [unwired: 1 in]
              }
              event "_InterfaceFolderSuffix", "TriggerSuffixChange": Value Change {
                n190 = event-data() -> ("OldVal"=w361:string)  [unwired: 1 in]
                n191 = local read "_InterfaceName"() -> (w363:string)
                n192 = local read "_InterfaceFolder"() -> (w365:path)
                n193 = call "File_NewPathGeneartor.vi"("NewPath"=w365, "OldPath"=w365, "NewName"=w363, "OldName"=w363, "NewSuffix"="_InterfaceFolderSuffix", "OldSuffix"=w361) -> ("PathOut"=w364:path, "NameOut"=w359:string, "SuffixOut"=w360:string)  [unwired: 11 in]
                n194 = local write "_InterfaceName"(w359) -> ()
                n195 = local write "_InterfaceFolder"(w364) -> ()
                n196 = local write "_InterfaceFolderSuffix"(w360) -> ()
              }
              event "_InterfaceFolder": Value Change {
                n197 = event-data() -> ("OldVal"=w371:path)  [unwired: 1 in]
                n198 = local read "_InterfaceFolderSuffix"() -> (w368:string)
                n199 = local read "_InterfaceName"() -> (w373:string)
                n200 = call "File_NewPathGeneartor.vi"("NewPath"="_InterfaceFolder", "OldPath"=w371, "NewName"=w373, "OldName"=w373, "NewSuffix"=w368, "OldSuffix"=w368) -> ("PathOut"=w374:path, "NameOut"=w370:string, "SuffixOut"=w369:string)  [unwired: 11 in]
                n201 = local write "_InterfaceFolder"(w374) -> ()
                n202 = local write "_InterfaceName"(w370) -> ()
                n203 = local write "_InterfaceFolderSuffix"(w369) -> ()
              }
            }
            n204 = Bundle By Name(cluster=w218, "Cancel"=w234) -> (w232:T14)
          }
          frame "UpdateMethodsList" {
            w385 = ""
            n205 = local read "M"() -> (w389:string[][])
            n206 = for {
              tunnel: w389 -> [w407] mode=indexing
              tunnel: [w407] -> w387 mode=indexing if=w401
              shift-right: [w405] -> _
              shift-left: string[] [] -> [w399]
              n207 = Index Array(array=w407) -> (element=w404:string)  [unwired: 1 in]
              n208 = Empty String/Path?(string/path=w404) -> (empty?=w406:bool)
              n209 = Not(x=w406) -> (.not. x?=w400:bool)
              n210 = case shown="True" w400 {
                tunnel: w399 -> [w408 w411]
                tunnel: w404 -> [_ w410]
                tunnel: [w408 w409] -> w405
                frame False {
                }
                frame True {
                  n211 = Build Array (concatenate)(w411, w410) -> (w409:string[])
                }
              }
              n212 = Search 1D Array(1D array=w399, element=w404) -> (index of element=w403:i32)  [unwired: 1 in]
              n213 = Less Than 0?(x=w403) -> (x < 0?=w402:bool)
              n214 = Compound Arithmetic op=AND(w400, w402) -> (w401:bool)
            }
            n215 = local write "M"(w387) -> ()
            n216 = Matrix Size(0:w387) -> (1:w382:i32)  [unwired: 1 out]
            n217 = Initialize Array(w385, w382) -> (w377:string[])
            n218 = Initialize Array(1005 ("y"), w382) -> (w383:i32[])
            n219 = property on="Over" class="LstBox (strict)"("Item Names"=w377) -> ("Item Symbols"=w378:i32[])  [unwired: 2 in, 2 out]
            n220 = Build Array (concatenate)(w377, w385) -> (w381:string[])
            n221 = Build Array (concatenate)(w383, 1041 ("y")) -> (w380:i32[])
            n222 = property on="IconList" class="LstBox (strict)"("Item Names"=w381, "Item Symbols"=w380) -> ()  [unwired: 2 in, 2 out]
            n223 = for {
              tunnel: w378 -> [w395]
              tunnel: [w396] -> w379 mode=indexing
              tunnel: w377 -> [_] mode=indexing
              i -> [w394]
              n224 = Index Array(array=w395, index=w394) -> (element=w393:i32)
              n225 = case shown="37" w393 {
                tunnel: [38 37] -> w396
                frame 0, Default {
                }
                frame 37 {
                }
              }
            }
            n226 = property on="Over" class="LstBox (strict)"("Item Symbols"=w379) -> ()  [unwired: 2 in, 2 out]
          }
          frame "UpdateListDimensions" {
            n227 = property on="M" class="Tbl (strict)" props=["Height", "Height"]() -> ("Height"=w412:u32)  [unwired: 2 in, 3 out]
            n228 = property on="IconList" class="LstBox (strict)"("Height"=w412) -> ()  [unwired: 2 in, 2 out]
            n229 = property on="Over" class="LstBox (strict)"("Height"=w412) -> ()  [unwired: 2 in, 2 out]
          }
          frame "SaveChanges" {
            n230 = local read "_InterfaceFolderSuffix"() -> (w419:string)
            n231 = call "BaseProvider_IniFileSettings.vi"() -> ("IniFileSettings"=w417:T19)  [unwired: 18 in, 1 out]
            n232 = Bundle By Name(cluster=w417, "InterfaceFolderSuffix"=w419) -> (w418:T19)
            n233 = Not Equal?(x=w418, y=w417) -> (x != y?=w416:bool)
            n234 = case shown="True" w416 {
              tunnel: w418 -> [_ w423]
              frame False {
              }
              frame True {
                n235 = call "BaseProvider_IniFileSettings.vi"("IniFileSettings"=w423, "Action"=enum16{"Read", "Load", "Save"}."Save") -> ()  [unwired: 16 in, 2 out]
              }
            }
          }
          frame "Error", "Exit", Default {
          }
        }
      }
      n236 = call "GDSString_AddStatesToQueue.vi"() -> ()  [unwired: 15 in, 1 out]
    }
    frame Error {
    }
  }
  "Reference out" <- w45
  "error out" <- w47
  n237 = call "CommonVIs_ClassIconSelection.vi"("IconsToShow(All)"=CommonVIs_ClassIconSelection_Action."Only Interface", "Icon"=w22, "Messages(Stop or Empty string will stop this VI)"=w3, "IconSelection"=w21) -> ()  [unwired: 8 in]
  n238 = call "GDSString_PlaceHolderText.vi"("BooleanUserEventToStopPlaceHolderVI"=w3, "PlaceholderText"="Interface name filter" ("InterfaceFilter"), "PlaceholderTextFont(Grey,Italic)"=T9 {"Font Name"="", "Size"=0, "Bold"=FALSE, "Italic"=TRUE, "Underline"=FALSE, "Strikeout"=FALSE, "Color"=10329501}, "NormalTextFont(Black)"=T9 {"Font Name"="", "Size"=0, "Bold"=FALSE, "Italic"=FALSE, "Underline"=FALSE, "Strikeout"=FALSE, "Color"=0}, "PlaceholderStringRef"=w7) -> ()  [unwired: 6 in, 1 out]
  n239 = Generate User Event(user event=w19, event data cluster="Stop" ("Stop")) -> (user event out=w20:refnum<user-event>)  [unwired: 2 in, 1 out]
  n240 = Destroy User Event(user event=w20) -> ()  [unwired: 1 in, 1 out]
  n241 = control-ref of="Wire Style"() -> (w2:refnum<vi>)
  n242 = control-ref of="WireSelectionList"() -> (w1:refnum<vi>)
  n243 = call "CommonVIs_ClassWireSelection.vi"("Offset(-300,0)"=T8 {"Left"=-115, "Top"=18}, "SelectedWireStyle"=w2, "Messages(Stop or Empty string will stop this VI)"=w3, "WireSelectionList"=w1) -> ()  [unwired: 7 in, 1 out]
  n244 = stacked-sequence {
    tunnel: w43 -> [w437]
    tunnel: [w445] -> w42
    tunnel: [w444] -> w41
    tunnel: [w443] -> w40
    tunnel: [w442] -> w39
    tunnel: [w441] -> _
    tunnel: w16 -> [w438]
    tunnel: w38 -> [_]
    tunnel: [w436] -> w37
    tunnel: [w435] -> w12
    tunnel: [w434] -> w11
    frame #0 {
      n245 = Unbundle By Name(w437) -> ("Cancel"=w445:bool, "DeriveFromClassRef"=w440:refnum<vi>, "ParentInterfaces"=w434:path[])
      n246 = local read "_InterfaceFolder"() -> (w444:path)
      n247 = local read "_InterfaceName"() -> (w443:string)
      n248 = local read "_InterfaceFolderSuffix"() -> (w436:string)
      n249 = property on="Over" class="LstBox (strict)"() -> ("Item Symbols"=w433:i32[])  [unwired: 2 in, 2 out]
      n250 = local read "_ClassDescription"() -> (w442:string)
      n251 = local read "M"() -> (w432:string[][])
      n252 = for {
        tunnel: w432 -> [w459] mode=indexing
        tunnel: [w455] -> w435 mode=indexing if=w446
        tunnel: w433 -> [w451]
        i -> [w450]
        n253 = Index Array(array=w459) -> (element #1=w457:string, element #2=w456:string)  [unwired: 2 in]
        n254 = Index Array(array=w451, index=w450) -> (element=w449:i32)
        n255 = call <vilib>:"Trim Whitespace.vi"("string"=w457) -> ("trimmed string"=w453:string)  [unwired: 1 in]
        n256 = call <vilib>:"Trim Whitespace.vi"("string"=w456) -> ("trimmed string"=w454:string)  [unwired: 1 in]
        n257 = Not Equal?(x=w449, y=37) -> (x != y?=w447:bool)
        n258 = Bundle By Name(cluster=T4 {"Name"="", "Description"="", "MethodsArgumentsIn"=[], "MethodsArgumentsOut"=[], "DecendantsMustOverride"=FALSE} ("MethodToCreate"), "Name"=w453, "Description"=w454, "DecendantsMustOverride"=w447) -> (w455:T4)
        n259 = Empty String/Path?(string/path=w453) -> (empty?=w452:bool)
        n260 = Not(x=w452) -> (.not. x?=w446:bool)
      }
      n261 = Not Equal?(x=w440, y=w438) -> (x != y?=w439:bool)
      n262 = case shown="True" w439 {
        tunnel: [_ w461] -> w441
        tunnel: w440 -> [_ w460]
        frame False {
        }
        frame True {
          n263 = Close Reference(reference=w460) -> (error out=w461:errorcluster)  [unwired: 1 in]
        }
      }
    }
  }
  "Cancelled" <- w42
  n264 = Bundle By Name(cluster=T3 {"InterfaceName"="", "InterfaceFolder"=path "", "InterfaceDescription"="", "FolderSuffix"="", "MethodsToCreate"=[], "ParentInterfaces"=[]} ("CreateInterfaceData"), "InterfaceFolder"=w41, "InterfaceName"=w40, "InterfaceDescription"=w39, "FolderSuffix"=w37, "MethodsToCreate"=w12, "ParentInterfaces"=w11) -> (→"CreateInterfaceData":T3)
